vi "UMLEditor GettingStartedDialog.vi"   [LabVIEW 2020]
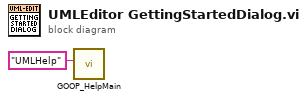
[diagram p0: block diagram]
diagram:
  n1 = call <resource>:"GOOP_HelpMain.vi"("File"="UMLHelp") -> ()  [unwired: 11 in]
